vi "Register.vi"(0 "BroadcastRegistry In":T2, 5 "Broadcast":string="status", 7 "SourceCSM":string="source", 9 "Name":string="api", 11 "TargetCSM":string="target", 12 "Register Type":T1=enum."Status") -> (4 "BroadcastRegistry Out":T2)   [LabVIEW 2017, in "Communicable State Machine.lvlib"]
doc: "### Register.vi\n\n-- <b>Controls</b> --\n- <b>BroadcastRegistry in</b>:\n- <b>status</b>:\n- <b>source</b>:\n- <b>api</b>:\n- <b>target</b>:\n\n-- <b>Indicators</b> --\n- <b>BroadcastRegistry out</b>:"
uses:
  Communicable State Machine.lvlib
  BroadcastRegistry.ctl
  AdvanceAPI/CSM - Broadcast Message Type.ctl
  BroadcastRegistry-Value.ctl
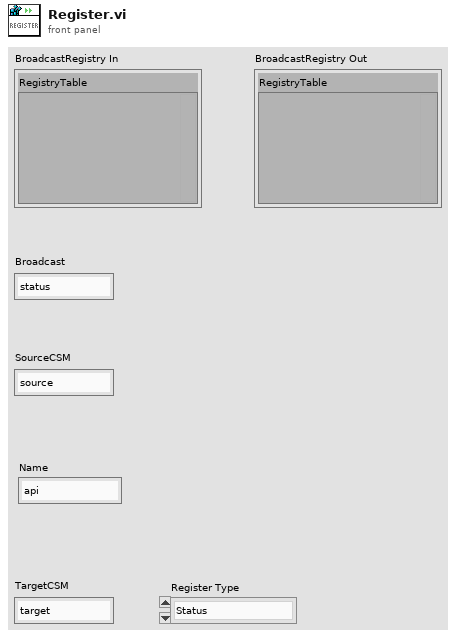
[diagram p1: front panel]
types:
  T1 = typedef "Communicable State Machine.lvlib/CSM - Broadcast Message Type.ctl" = enum16{"<Null>", "Status", "Interrupt"}
  T2 = typedef "Communicable State Machine.lvlib/BroadcastRegistry.ctl" = cluster{"RegistryTable":variant}
  T3 = typedef "Communicable State Machine.lvlib/BroadcastRegistry-Value.ctl" = cluster{"Name":string, "Register Type":T1}
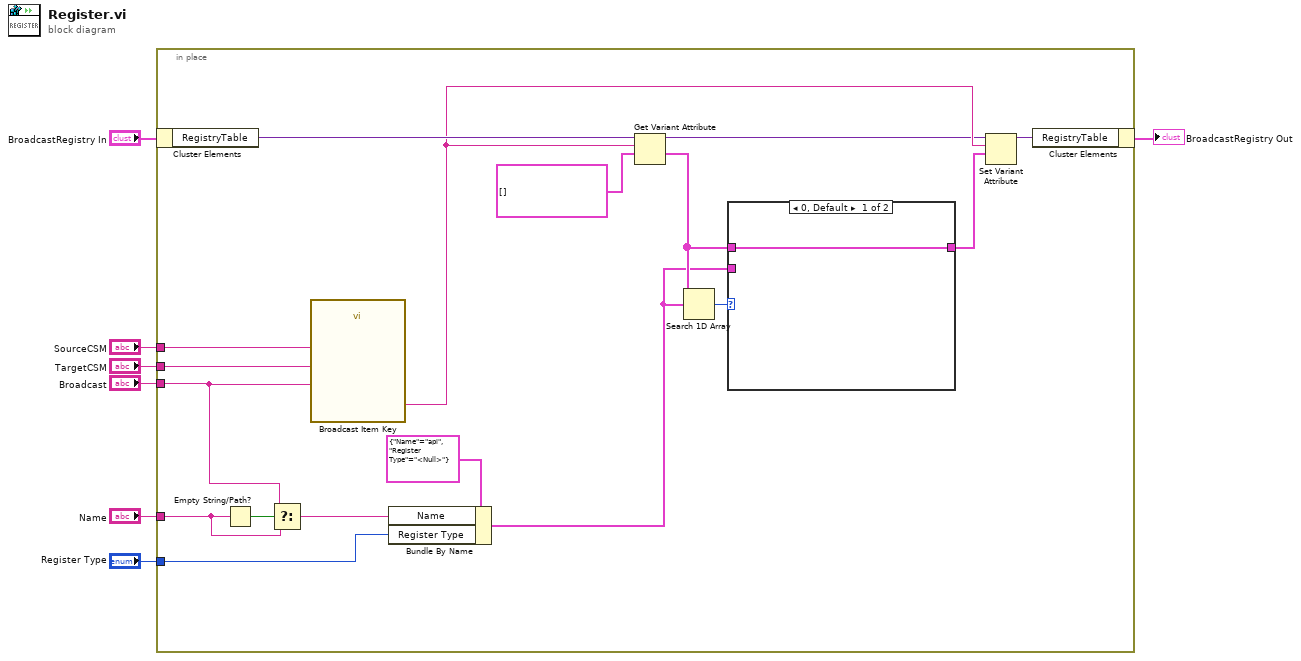
[diagram p0: block diagram]
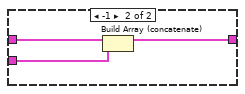
[diagram p2: hidden frame]
diagram:
  n1 = in-place {
    in-place-border: "Broadcast" -> [w12]
    in-place-border: "TargetCSM" -> [w23]
    in-place-border: "SourceCSM" -> [w22]
    in-place-border: "Name" -> [w21]
    in-place-border: "Register Type" -> [w9]
    n2 = in-place-cluster #1("BroadcastRegistry In") -> ("RegistryTable"=w20:variant)
    n3 = Empty String/Path?(string/path=w21) -> (empty?=w24:bool)
    n4 = Select(t=w12, s=w24, f=w21) -> (s? t:f=w10:string)
    n5 = call "Broadcast Item Key.vi"("Status"=w12, "Target"=w23, "Source"=w22) -> ("Key"=w19:string)  [unwired: 2 in]
    n6 = Bundle By Name(cluster=T3 {"Name"="api", "Register Type"=enum."<Null>"}, "Name"=w10, "Register Type"=w9) -> (w8:T3)
    n7 = Get Variant Attribute(Variant=w20, name=w19, default value (empty Variant)=T3[] [] ("output cluster")) -> (duplicate Variant=w16:variant, value=w14:T3[])  [unwired: 1 in, 2 out]
    n8 = Search 1D Array(1D array=w14, element=w8) -> (index of element=w17:i32)  [unwired: 1 in]
    n9 = case shown="0, Default" w17 {
      tunnel: w14 -> [w25 w28]
      tunnel: [w25 w27] -> w13
      tunnel: w8 -> [_ w26]
      frame 0, Default {
      }
      frame -1 {
        n10 = Build Array (concatenate)(w28, w26) -> (w27:T3[])
      }
    }
    n11 = Set Variant Attribute(Variant=w16, name=w19, value=w13) -> (Variant out=w18:variant)  [unwired: 1 in, 2 out]
    n12 = in-place-cluster #1("RegistryTable"=w18) -> (→"BroadcastRegistry Out":T2)
  }
